vi "Complete Handler Result.vi"(8 "error in":errorcluster, 9 "serverInfo":string, 10 "method":string, 11 "handler response":string) -> (0 "error out":errorcluster, 3 "response":string)   [LabVIEW 2020, in "MCP Server.lvlib"]
doc: "Completes the handler's answer to a modern (MCP 2026-07-28) request that is not server/discover and did not ask the user: a response with a result gets the result fields (Add Result Fields.vi); any other response goes through Remap Resource Not Found.vi. Used by Complete Modern MCP Result.vi.\n\nRuns regardless of error in, which is passed through unchanged; the JSONtext errors are not passed on."
uses:
  MCP Server.lvlib
  <vilib>/JDP Science/JSONtext/Next JSON Value.vi
  <vilib>/JDP Science/JSONtext/String Subset.vi
  <vilib>/JDP Science/JSONtext/Parsing/Advance past next JSON Value (inlined COPY).vi
  <vilib>/JDP Science/JSONtext/Parsing/Advance past whitespace.vi
  <vilib>/JDP Science/JSONtext/Parsing/Advance past String.vi
  <vilib>/JDP Science/JSONtext/Parsing/Advance past Number.vi
  <vilib>/JDP Science/JSONtext/Parsing/Advance past Line Ending.vi
  <vilib>/JDP Science/JSONtext/Parsing/Parse Full Path or Item Name.vi
  <vilib>/JDP Science/JSONtext/Parsing/Advance past Array.vi
  <vilib>/JDP Science/JSONtext/Parsing/Advance past Object.vi
  <vilib>/JDP Science/JSONtext/support/Error Cluster From Code.vi
  <vilib>/JDP Science/JSONtext/Offset/Find Item Locations by Path.vi
  <vilib>/JDP Science/JSONtext/JSONtext.lvlib
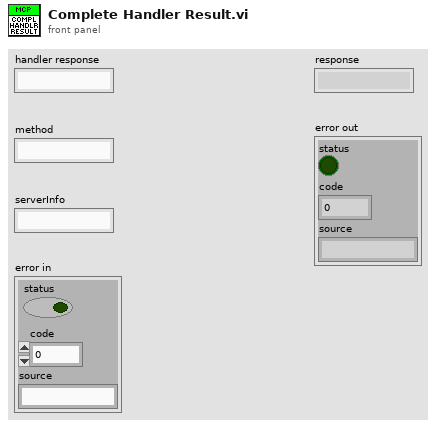
[diagram p1: front panel]
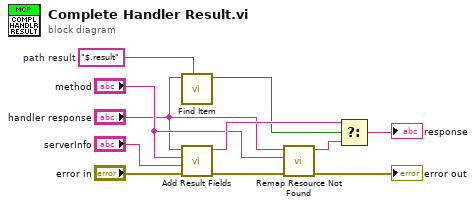
[diagram p0: block diagram]
diagram:
  w5 = "$.result"  # path result
  n1 = call <vilib>:"Find Item.vi"("$Path or Item Name"=w5, "JSON"="handler response") -> ("Found"=w6:bool)  [unwired: 6 in, 3 out]
  n2 = call "Add Result Fields.vi"("error in"="error in", "serverInfo"="serverInfo", "method"="method", "response"="handler response") -> ("error out"=w8:errorcluster, "response out"=w7:string)  [unwired: 6 in]
  n3 = call "Remap Resource Not Found.vi"("error in"=w8, "method"="method", "response"="handler response") -> ("error out"=→"error out":errorcluster, "response out"=w9:string)  [unwired: 7 in]
  n4 = Select(t=w7, s=w6, f=w9) -> (s? t:f=→"response":string)
